vi "Module Cleanup.vi"(8 "error in (no error)":errorcluster, 11 "ValveControlModule in":refnum<class "DigitalControlModule.lvclass">) -> (0 "error out":errorcluster, 3 "ValveControlModule out":refnum<class "DigitalControlModule.lvclass">)   [LabVIEW 2020, in "VolatusControl.lvlib" / "DigitalControlModule.lvclass"]
uses:
  DigitalControlModule.lvclass
  DigitalControlModule.lvclass/DigitalControlModule.ctl
  VolatusData/Data Buffer DBL/Data Buffer DBL.lvclass
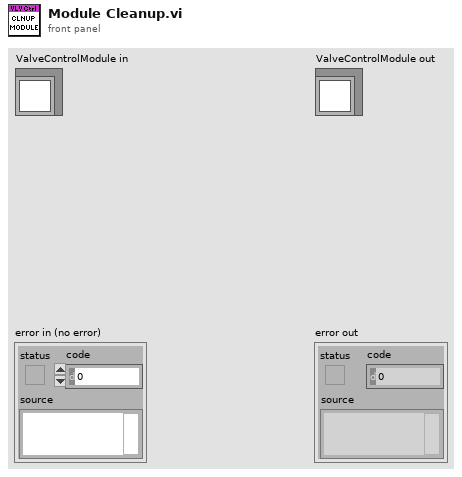
[diagram p1: front panel]
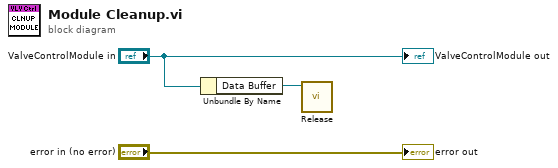
[diagram p0: block diagram]
diagram:
  n1 = Unbundle By Name("ValveControlModule in") -> ("Data Buffer"=w1:refnum<class "Data Buffer DBL.lvclass">)
  n2 = call "Release.vi"("Data Buffer in"=w1) -> ()  [unwired: 10 in, 1 out]
  "error out" <- "error in (no error)"
  "ValveControlModule out" <- "ValveControlModule in"
